vi "work2_Cooker Module.vi"() -> ()   [LabVIEW 2020]
panel:
  out "Cooked today":string[](array[string])
  in  "Nb":i16
  in  "Burgers":bool
  in  "Meal":bool
  in  "stop":bool
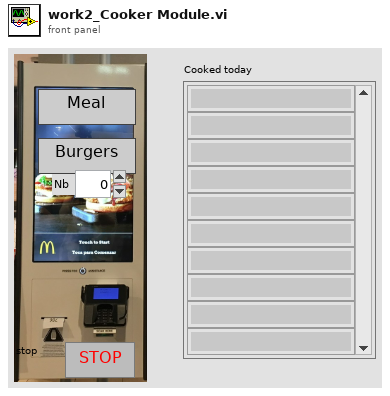
[diagram p1: front panel]
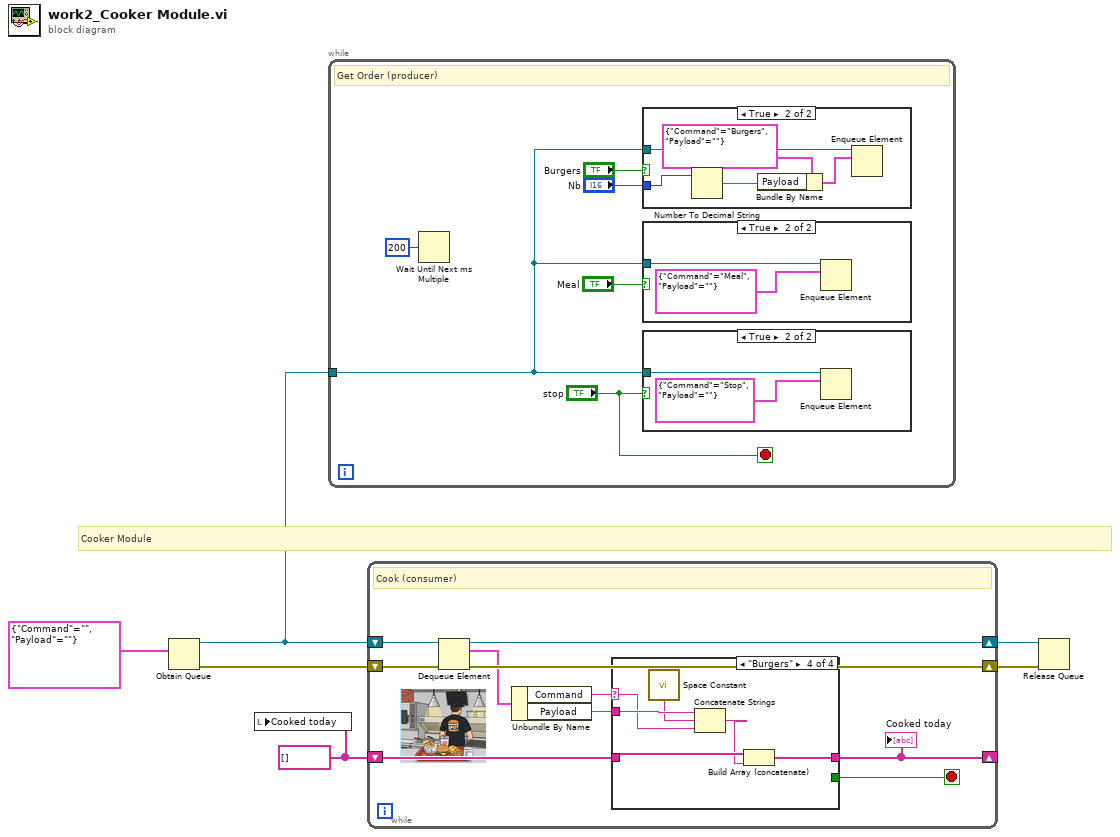
[diagram p0: block diagram]
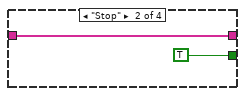
[diagram p6: hidden frame]
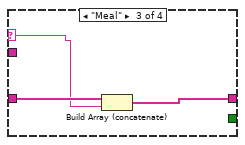
[diagram p7: hidden frame]
diagram:
  w1 = string[] [] ("Cooked today")
  # "Cooker Module"
  n1 = Obtain Queue(element data type=cluster{"Command":string, "Payload":string} {"Command"="", "Payload"=""}) -> (queue out=w3:refnum<queue>, error out=w6:errorcluster)  [unwired: 4 in, 1 out]
  n2 = local write "Cooked today"(w1) -> ()
  n3 = while {
    tunnel: w3 -> [w8]
    stop <- "stop" stop-if-true
    # "Get Order (producer)"
    n4 = Wait Until Next ms Multiple(millisecond multiple=u32 200) -> ()  [unwired: 1 out]
    n5 = case shown="True" "Burgers" {
      tunnel: w8 -> [_ w17]
      tunnel: "Nb" -> [_ w14]
      frame False {
      }
      frame True {
        n6 = Number To Decimal String(number=w14) -> (decimal integer string=w13:string)  [unwired: 1 in]
        n7 = Bundle By Name(cluster=cluster{"Command":string, "Payload":string} {"Command"="Burgers", "Payload"=""} ("element"), "Payload"=w13) -> (w15:cluster{"Command":string, "Payload":string})
        n8 = Enqueue Element(queue=w17, element=w15) -> ()  [unwired: 2 in, 3 out]
      }
    }
    n9 = case shown="True" "Meal" {
      tunnel: w8 -> [_ w19]
      frame False {
      }
      frame True {
        n10 = Enqueue Element(queue=w19, element=cluster{"Command":string, "Payload":string} {"Command"="Meal", "Payload"=""}) -> ()  [unwired: 2 in, 3 out]
      }
    }
    n11 = case shown="True" "stop" {
      tunnel: w8 -> [_ w21]
      frame False {
      }
      frame True {
        n12 = Enqueue Element(queue=w21, element=cluster{"Command":string, "Payload":string} {"Command"="Stop", "Payload"=""}) -> ()  [unwired: 2 in, 3 out]
      }
    }
  }
  n13 = while {
    shift-right: [w29] -> w4
    shift-left: w6 -> [w31]
    shift-right: [w30] -> w5
    shift-left: w3 -> [w28]
    shift-right: [w23] -> _
    shift-left: w1 -> [w24]
    stop <- w25 stop-if-true
    # "Cook (consumer)"
    n14 = Dequeue Element(queue=w28, error in (no error)=w31) -> (queue out=w30:refnum<queue>, element=w27:cluster{"Command":string, "Payload":string}, error out=w29:errorcluster)  [unwired: 1 in, 1 out]
    n15 = Unbundle By Name(w27) -> ("Command"=w26:string, "Payload"=w22:string)
    n16 = case shown="\"Burgers\"" w26 {
      selector: w26 -> [_ _ w35 w40]
      tunnel: [_ TRUE _ _] -> w25
      tunnel: w24 -> [w32 w33 w37 w42]
      tunnel: [w32 w33 w36 w43] -> w23
      tunnel: w22 -> [_ _ _ w41]
      frame Default {
      }
      frame "Stop" {
      }
      frame "Meal" {
        n17 = Build Array (concatenate)(w37, w35) -> (w36:string[])
      }
      frame "Burgers" {
        n18 = call <vilib>:"Space Constant.vi"() -> ("String"=w39:string)
        n19 = Concatenate Strings(w41, w39, w40) -> (w38:string)
        n20 = Build Array (concatenate)(w42, w38) -> (w43:string[])
      }
    }
    "Cooked today" <- w23
  }
  n21 = Release Queue(queue=w5, error in (no error)=w4) -> ()  [unwired: 1 in, 3 out]
